vi "ziGetEventBoxcarVector.vi"(8 "Error In":errorcluster, 11 "Handle In":T2 {"Handle" format="0x%08x"; "Conn" format="0x%08x"}) -> (0 "Error Out":errorcluster, 3 "Handle Out":T2 {"Handle" format="0x%08x"; "Conn" format="0x%08x"})   [LabVIEW 2009, in "Zurich Instruments LabOne.lvlib"]
uses:
  <instrlib>/Zurich Instruments LabOne/Zurich Instruments LabOne.lvlib
  <instrlib>/Zurich Instruments LabOne/Public/ziTypeHandle.ctl
  <instrlib>/Zurich Instruments LabOne/Public/Data/ziTypeBoxcarVector.ctl
  <instrlib>/Zurich Instruments LabOne/Private/ziLV64.dll
panel:
  in  "Boxcar Vector In":T1
  out "Boxcar Vector Out":T1
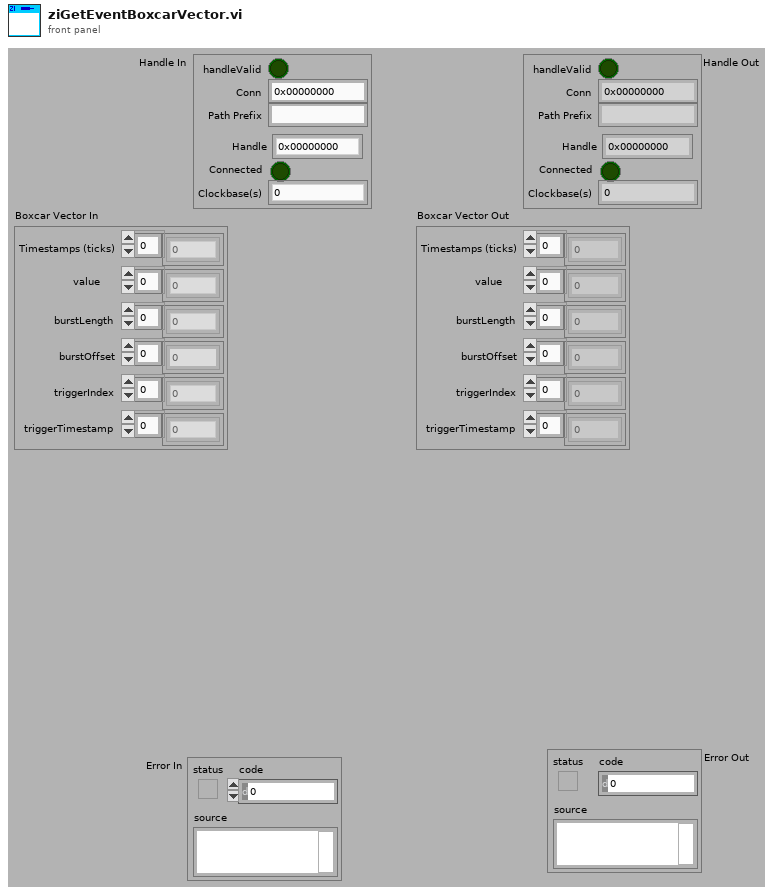
[diagram p1: front panel]
types:
  T1 = typedef "Zurich Instruments LabOne.lvlib/ziTypeBoxcarVector.ctl" = cluster{"Timestamps (ticks)":u64[], "value":dbl[], "burstLength":u32[], "burstOffset":u32[], "triggerIndex":u32[], "triggerTimestamp":u64[]}
  T2 = typedef "Zurich Instruments LabOne.lvlib/ziTypeHandle.ctl" = cluster{"handleValid":bool, "Conn":u64, "Path Prefix":string, "Handle":u64, "Connected":bool, "Clockbase(s)":dbl}
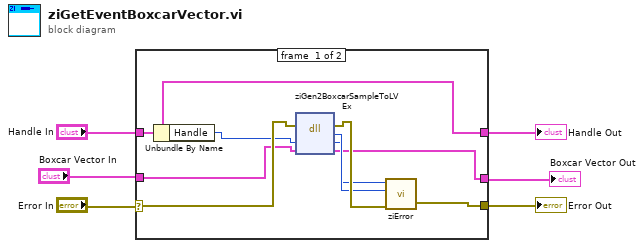
[diagram p0: block diagram]
diagram:
  n1 = case shown="No Error" "Error In" {
    selector: "Error In" -> [w13 w17]
    tunnel: "Handle In" -> [w14 w18]
    tunnel: [w14 w18] -> w5
    tunnel: [w15 w17] -> w4
    tunnel: [w7 w16] -> w2
    tunnel: "Boxcar Vector In" -> [w11 w16]
    frame #0 {
      n2 = Unbundle By Name(w14) -> ("Handle"=w12:u64)
      n3 = dll-call lib="C:/Program Files/National Instruments/LabVIEW 2009/instr.lib/Zurich Instruments LabOne/Private/ziLV*.*" fn="ziGen2BoxcarSampleToLVEx"(error in=w13, "ziEventBuffer"=w12, "BoxcarSample"=w11) -> (error out=w10:errorcluster, "return type"=w9:u32, "ziEventBuffer"=w8:u64, "BoxcarSample"=w7:T1)  [unwired: 2 in, 1 out]
      n4 = call <instrlib>:"ziError.vi"("Conn"=w8, "ziErrorCode"=w9, "Error In"=w10) -> ("Error Out"=w15:errorcluster)  [unwired: 2 in, 1 out]
    }
    frame #1 {
    }
  }
  "Handle Out" <- w5
  "Error Out" <- w4
  "Boxcar Vector Out" <- w2
